vi "CSMOMgr-Delete CSMO.vi"(8 "Error In":errorcluster caption="error in (no error)", 10 "Queue Name":string, 11 "CSMOMgr":T1) -> (0 "error out":errorcluster, 2 "#left":i32, 3 "CSMOMgr Out":T1)   [LabVIEW 2017, in "Communicable State Machine.lvlib"]
uses:
  Communicable State Machine.lvlib
  Def-CSMOMgr.ctl
  FGV-BroadcastRegistry/Operation-BroadcastRegistry.ctl
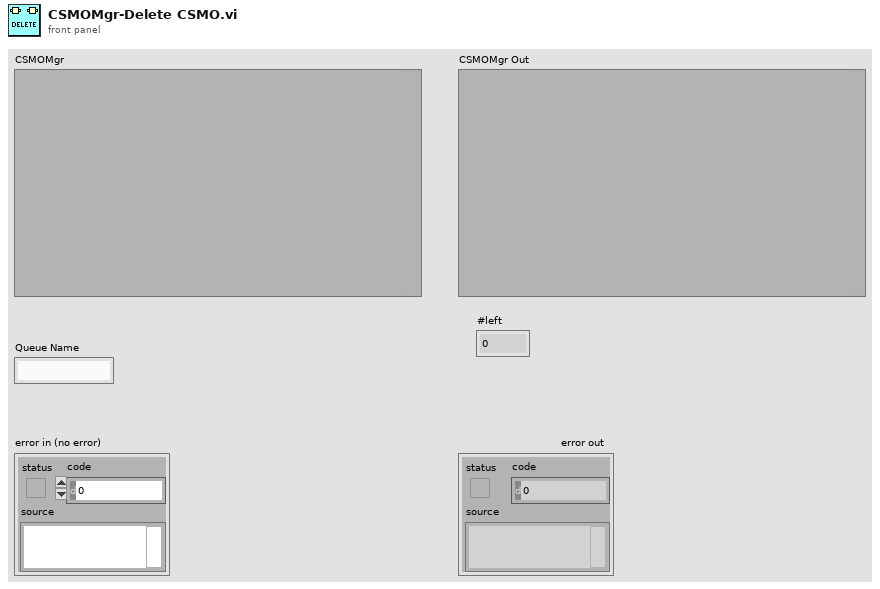
[diagram p1: front panel]
types:
  T1 = typedef "Communicable State Machine.lvlib/Def-CSMOMgr.ctl" = variant
  T2 = typedef "Communicable State Machine.lvlib/_CSMObj.ctl" = cluster{"info":T3, "Refs":T5}
  T3 = typedef "Communicable State Machine.lvlib/_CSMObj-Info.ctl" = cluster{"Module Name":string, "Requested Name":string, "Group Name":string, "Mode":T4, "Allowed Messages":string[]}
  T4 = typedef "Communicable State Machine.lvlib/_CSM_MODE.ctl" = enum16{"Not Exist", "Stand Alone", "CSM", "Worker", "Worker Agent", "Chain Node", "Chain"}
  T5 = typedef "Communicable State Machine.lvlib/_CSMObj-Refs.ctl" = cluster{"WatchDogQ":refnum<queue>, "CSMDataDVR":refnum<data-value>, "Queue":T6, "GroupDataDVR":refnum<data-value>, "TagMap":refnum<data-value>, "ExitEvent":refnum<user-event>, "NewStateEvent":refnum<user-event>, "StatusEvent":refnum<user-event>, "InterruptEvent":refnum<user-event>}
  T6 = typedef "Communicable State Machine.lvlib/Priority Queue.ctl" = cluster{"HPriorityQ":refnum<queue>, "LowPriorityQ":refnum<queue>}
  T7 = typedef "Communicable State Machine.lvlib/Operation-BroadcastRegistry.ctl" = enum16{"Delete Source Module", "Delete Target Module", "Remove Module", "Register", "Unregister", "Check", "List Status", "List Entries", "List Status Of Source", "Drop", "Register As Status", "Register As Interrupt"}
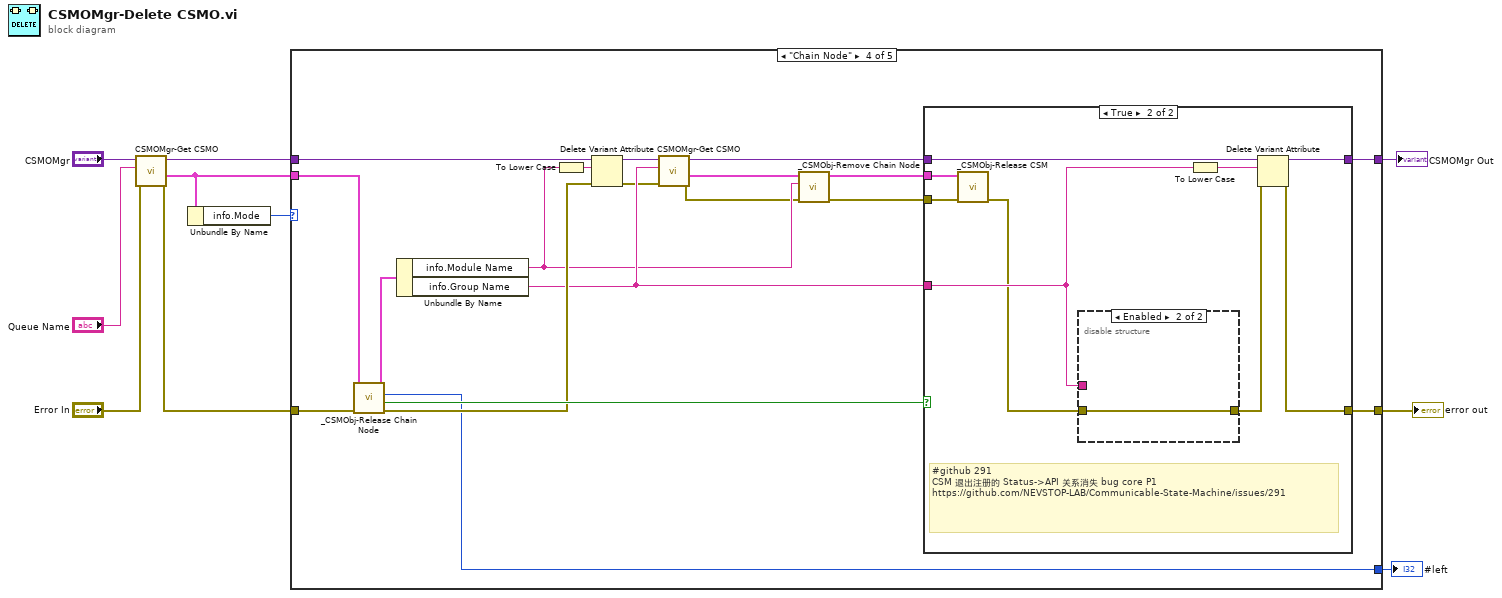
[diagram p0: block diagram]
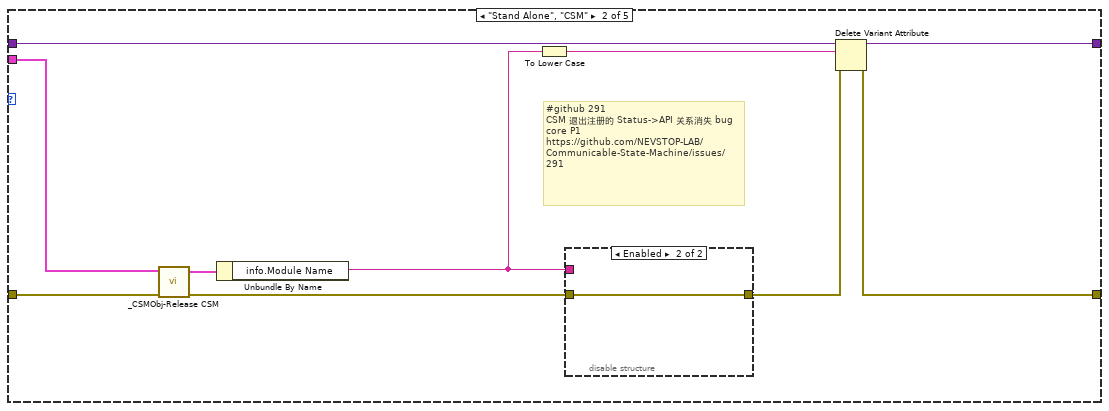
[diagram p3: hidden frame]
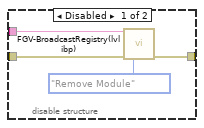
[diagram p4: hidden frame]
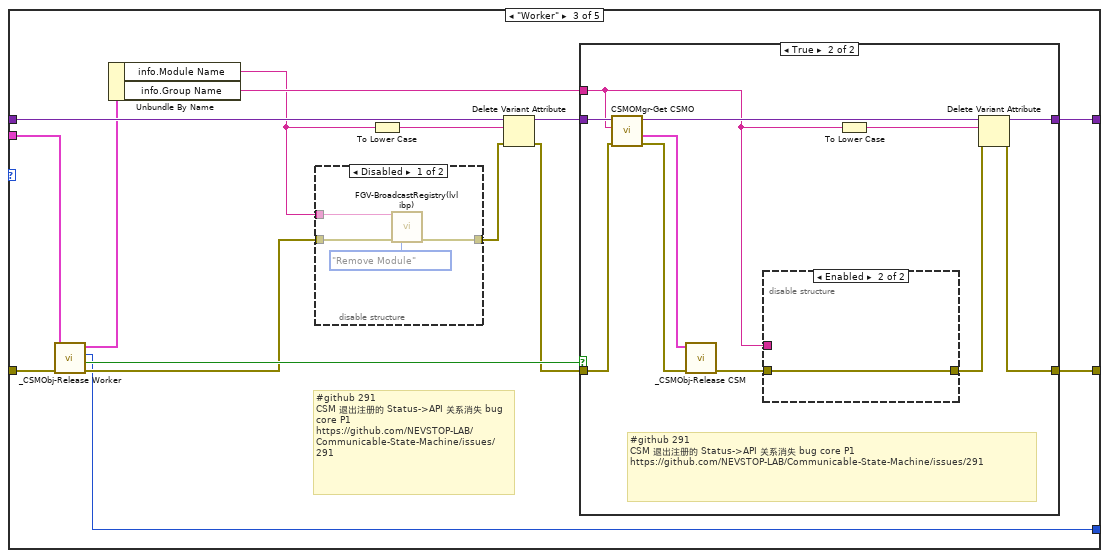
[diagram p5: hidden frame]
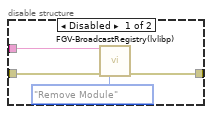
[diagram p8: hidden frame]
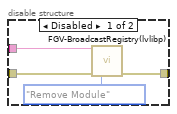
[diagram p10: hidden frame]
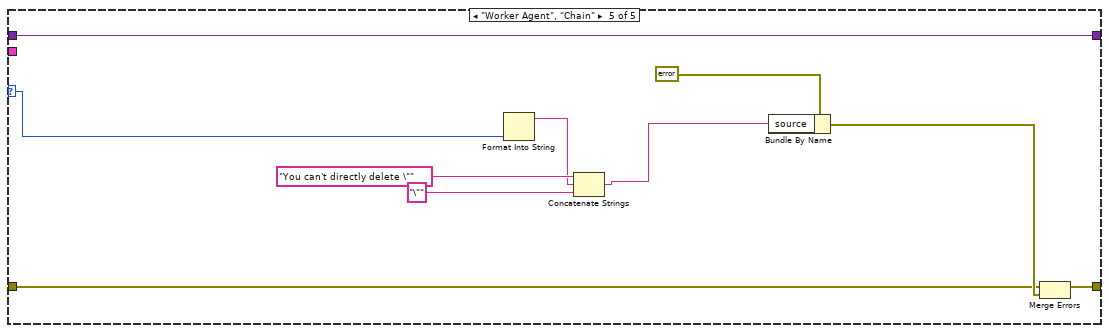
[diagram p11: hidden frame]
diagram:
  n1 = call "CSMOMgr-Get CSMO.vi"("Error In"="Error In", "Queue Name"="Queue Name", "CSMOMgr"="CSMOMgr") -> ("error out"=w10:errorcluster, "Values"=w8:T2, "CSMOMgr Out"=w9:T1)  [unwired: 5 in, 1 out]
  n2 = Unbundle By Name(w8) -> ("info.Mode"=w7:T4)
  n3 = case shown="\"Chain Node\"" w7 {
    selector: w7 -> [_ _ _ _ w101]
    tunnel: [w12 w22 w42 w84 w110] -> w3
    tunnel: [w11 w21 w41 w83 w104] -> w2
    tunnel: w8 -> [_ w20 w40 w82 _]
    tunnel: w10 -> [w11 w19 w38 w80 w103]
    tunnel: w9 -> [w12 w18 w37 w76 w110]
    tunnel: [_ _ w28 w66 _] -> w1
    frame "Not Exist", Default {
    }
    frame "Stand Alone", "CSM" {
      # "#github 291\nCSM 退出注册的 Status->API 关系消失 bug core P1\nhttps://github.com/NEVSTOP-LAB/Communicable-State-Machine/issues/291"
      n4 = call "_CSMObj-Release CSM.vi"("Error In"=w19, "CSMQ In"=w20) -> ("error out"=w16:errorcluster, "CSMQ Out"=w17:T2)  [unwired: 7 in, 1 out]
      n5 = Unbundle By Name(w17) -> ("info.Module Name"=w14:string)
      n6 = To Lower Case(string=w14) -> (all lower case string=w13:string)
      n7 = disable-structure shown="Enabled" {
        disable-tunnel: w16 -> [w26 w27]
        disable-tunnel: [w25 w27] -> w15
        disable-tunnel: w14 -> [w24 _]
        frame Disabled {
          n8 = call "FGV-BroadcastRegistry(lvlibp).vi"("Source"=w24, "Error In"=w26, "Operation"=Operation-BroadcastRegistry."Remove Module") -> ("error out"=w25:errorcluster)  [unwired: 10 in, 2 out]
        }
        frame Enabled {
        }
      }
      n9 = Delete Variant Attribute(4:w15, 6:w13, 7:w18) -> (0:w21:errorcluster, 3:w22:variant)  [unwired: 1 out]
    }
    frame "Worker" {
      # "#github 291\nCSM 退出注册的 Status->API 关系消失 bug core P1\nhttps://github.com/NEVSTOP-LAB/Communicable-State-Machine/issues/291"
      n10 = call "_CSMObj-Release Worker.vi"("Error In"=w38, "CSMQ In"=w40) -> ("error out"=w31:errorcluster, "Group Release?"=w39:bool, "#left"=w28:i32, "CSMQ Out"=w34:T2)  [unwired: 6 in]
      n11 = Unbundle By Name(w34) -> ("info.Module Name"=w30:string, "info.Group Name"=w33:string)
      n12 = disable-structure shown="Disabled" {
        disable-tunnel: [w45 w47] -> w32
        disable-tunnel: w31 -> [w44 w47]
        disable-tunnel: w30 -> [w43 _]
        frame Disabled {
          n13 = call "FGV-BroadcastRegistry(lvlibp).vi"("Source"=w43, "Error In"=w44, "Operation"=Operation-BroadcastRegistry."Remove Module") -> ("error out"=w45:errorcluster)  [unwired: 10 in, 2 out]
        }
        frame Enabled {
        }
      }
      n14 = To Lower Case(string=w30) -> (all lower case string=w29:string)
      n15 = Delete Variant Attribute(4:w32, 6:w29, 7:w37) -> (0:w35:errorcluster, 3:w36:variant)  [unwired: 1 out]
      n16 = case shown="True" w39 {
        tunnel: w33 -> [_ w53]
        tunnel: w36 -> [w49 w55]
        tunnel: [w49 w60] -> w42
        tunnel: w35 -> [w48 w52]
        tunnel: [w48 w58] -> w41
        frame False {
        }
        frame True {
          # "#github 291\nCSM 退出注册的 Status->API 关系消失 bug core P1\nhttps://github.com/NEVSTOP-LAB/Communicable-State-Machine/issues/291"
          n17 = call "CSMOMgr-Get CSMO.vi"("Error In"=w52, "Queue Name"=w53, "CSMOMgr"=w55) -> ("error out"=w50:errorcluster, "Values"=w51:T2, "CSMOMgr Out"=w54:T1)  [unwired: 5 in, 1 out]
          n18 = call "_CSMObj-Release CSM.vi"("Error In"=w50, "CSMQ In"=w51) -> ("error out"=w56:errorcluster)  [unwired: 7 in, 2 out]
          n19 = disable-structure shown="Enabled" {
            disable-tunnel: [w63 w65] -> w59
            disable-tunnel: w56 -> [w62 w65]
            disable-tunnel: w53 -> [w61 _]
            frame Disabled {
              n20 = call "FGV-BroadcastRegistry(lvlibp).vi"("Source"=w61, "Error In"=w62, "Operation"=Operation-BroadcastRegistry."Remove Module") -> ("error out"=w63:errorcluster)  [unwired: 10 in, 2 out]
            }
            frame Enabled {
            }
          }
          n21 = To Lower Case(string=w53) -> (all lower case string=w57:string)
          n22 = Delete Variant Attribute(4:w59, 6:w57, 7:w54) -> (0:w58:errorcluster, 3:w60:variant)  [unwired: 1 out]
        }
      }
    }
    frame "Chain Node" {
      n23 = call "_CSMObj-Release Chain Node.vi"("Error In"=w80, "CSMQ In"=w82) -> ("error out"=w79:errorcluster, "Group Release?"=w81:bool, "#left"=w66:i32, "CSMQ Out"=w78:T2)  [unwired: 6 in]
      n24 = Unbundle By Name(w78) -> ("info.Module Name"=w71:string, "info.Group Name"=w77:string)
      n25 = To Lower Case(string=w71) -> (all lower case string=w68:string)
      n26 = Delete Variant Attribute(4:w79, 6:w68, 7:w76) -> (0:w73:errorcluster, 3:w75:variant)  [unwired: 1 out]
      n27 = call "CSMOMgr-Get CSMO.vi"("Error In"=w73, "Queue Name"=w77, "CSMOMgr"=w75) -> ("error out"=w70:errorcluster, "Values"=w72:T2, "CSMOMgr Out"=w74:T1)  [unwired: 5 in, 1 out]
      n28 = call "_CSMObj-Remove Chain Node.vi"("Error In"=w70, "Requested Name"=w71, "CSMObj In"=w72) -> ("error out"=w69:errorcluster, "CSMObj Out"=w67:T2)  [unwired: 7 in]
      n29 = case shown="True" w81 {
        tunnel: w77 -> [_ w93]
        tunnel: w74 -> [w86 w95]
        tunnel: [w86 w94] -> w84
        tunnel: w69 -> [w85 w88]
        tunnel: [w85 w91] -> w83
        tunnel: w67 -> [_ w89]
        frame False {
        }
        frame True {
          # "#github 291\nCSM 退出注册的 Status->API 关系消失 bug core P1\nhttps://github.com/NEVSTOP-LAB/Communicable-State-Machine/issues/291"
          n30 = call "_CSMObj-Release CSM.vi"("Error In"=w88, "CSMQ In"=w89) -> ("error out"=w87:errorcluster)  [unwired: 7 in, 2 out]
          n31 = disable-structure shown="Enabled" {
            disable-tunnel: w93 -> [w98 _]
            disable-tunnel: [w97 w100] -> w92
            disable-tunnel: w87 -> [w96 w100]
            frame Disabled {
              n32 = call "FGV-BroadcastRegistry(lvlibp).vi"("Source"=w98, "Error In"=w96, "Operation"=Operation-BroadcastRegistry."Remove Module") -> ("error out"=w97:errorcluster)  [unwired: 10 in, 2 out]
            }
            frame Enabled {
            }
          }
          n33 = To Lower Case(string=w93) -> (all lower case string=w90:string)
          n34 = Delete Variant Attribute(4:w92, 6:w90, 7:w95) -> (0:w91:errorcluster, 3:w94:variant)  [unwired: 1 out]
        }
      }
    }
    frame "Worker Agent", "Chain" {
      n35 = Format Into String(w101) -> (resulting string=w102:string)  [unwired: 3 in, 1 out]
      n36 = Concatenate Strings("You can't directly delete \"" ("source"), w102, "\"" ("source")) -> (w106:string)
      n37 = Bundle By Name(cluster=errorcluster {"status"=TRUE, "code"=-1, "source"=""} ("error out"), "source"=w106) -> (w105:errorcluster)
      n38 = Merge Errors(w103, w105) -> (w104:errorcluster)
    }
  }
  "error out" <- w2
  "CSMOMgr Out" <- w3
  "#left" <- w1
